vi "dynamic_roi_setting.vi"(8 "right_line_center":i32, 9 "left_line_center":i32, 10 "mid_far Descriptor":T2={"Global Rectangle"=[475, 215, 533, 216], "Contours"=[{"ID"=enum."External", "Type"=2, "Coordinates"=[530, 210, 580, 210]}]} {"Contours"."Type" items=["No Selection", "Point", "Line", "Rectangle", "Oval", "Polygon", "Freehand Region", "Annulus", "Unused2", "Unused3", "Broken Line", "Freehand Line", "Rotated Rectangle"]}, 11 "mid_near Descriptor":T2={"Global Rectangle"=[475, 216, 344, 218], "Contours"=[{"ID"=enum."External", "Type"=2, "Coordinates"=[200, 210, 250, 210]}]} {"Contours"."Type" items=["No Selection", "Point", "Line", "Rectangle", "Oval", "Polygon", "Freehand Region", "Annulus", "Unused2", "Unused3", "Broken Line", "Freehand Line", "Rotated Rectangle"]}) -> (2 "far_roi":T1, 3 "near_roi":T1)   [LabVIEW 2024]
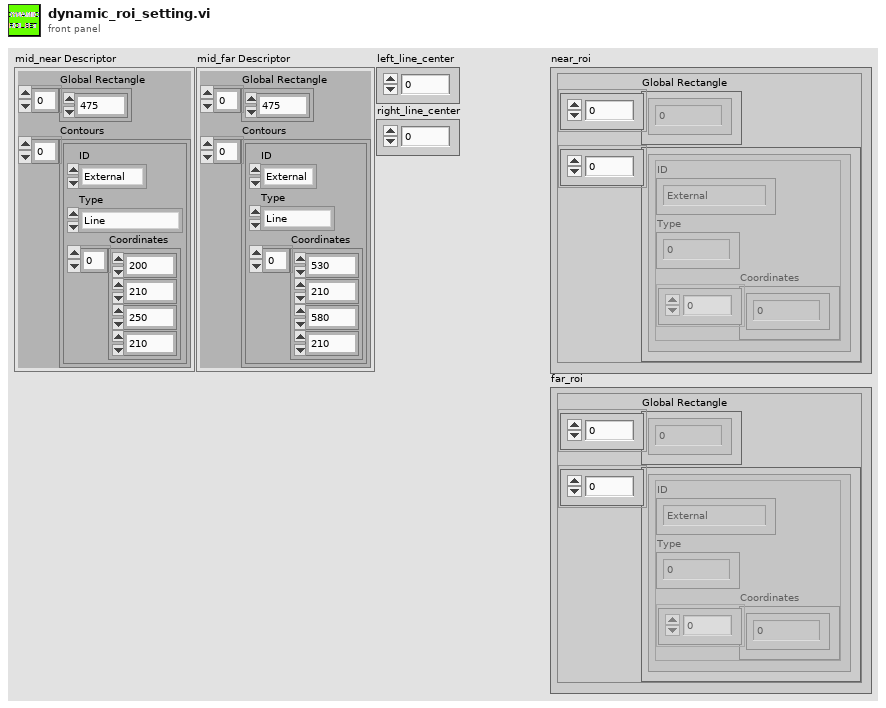
[diagram p1: front panel]
types:
  T1 = cluster{"Global Rectangle":i32[], "배열":cluster{"ID":enum32{"External", "Internal"}, "Type":u32, "Coordinates":i32[]}[]}
  T2 = cluster{"Global Rectangle":i32[], "Contours":cluster{"ID":enum32{"External", "Internal"}, "Type":u32, "Coordinates":i32[]}[]}
  T3 = cluster{"ID":enum32{"External", "Internal"}, "Type":u32, "Coordinates":i32[]}[]
  T4 = cluster{"ID":enum32{"External", "Internal"}, "Type":u32, "Coordinates":i32[]}
  T5 = cluster{"Global Rectangle":i32[], cluster{"ID":enum32{"External", "Internal"}, "Type":u32, "Coordinates":i32[]}[]}
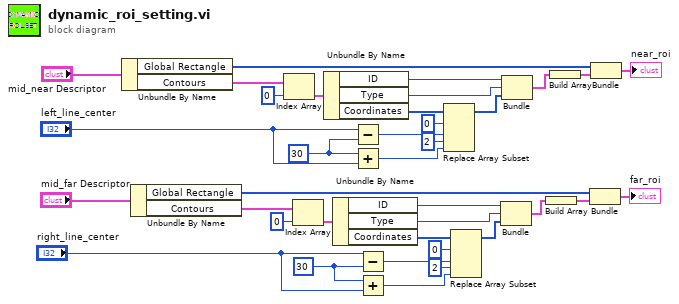
[diagram p0: block diagram]
diagram:
  w5 = 30
  w8 = 30
  n1 = Unbundle By Name("mid_near Descriptor") -> ("Global Rectangle"=w29:i32[], "Contours"=w36:T3)
  n2 = Unbundle By Name("mid_far Descriptor") -> ("Global Rectangle"=w18:i32[], "Contours"=w12:T3)
  n3 = Index Array(array=w36, index=0 ("인덱스")) -> (element=w34:T4)
  n4 = Index Array(array=w12, index=0 ("인덱스")) -> (element=w13:T4)
  n5 = Unbundle By Name(w34) -> ("ID"=w28:enum32{"External", "Internal"}, "Type"=w27:u32, "Coordinates"=w30:i32[])
  n6 = Unbundle By Name(w13) -> ("ID"=w19:enum32{"External", "Internal"}, "Type"=w20:u32, "Coordinates"=w17:i32[])
  n7 = Subtract(x="left_line_center", y=w8) -> (x-y=w7:i32)
  n8 = Add(x=w8, y="left_line_center") -> (x+y=w6:i32)
  n9 = Subtract(x="right_line_center", y=w5) -> (x-y=w4:i32)
  n10 = Add(x=w5, y="right_line_center") -> (x+y=w3:i32)
  n11 = Replace Array Subset(array=w30, new element #1=w7, index #1=0 ("인덱스"), new element #2=w6, index #2=2 ("인덱스")) -> (w26:i32[])
  n12 = Replace Array Subset(array=w17, new element #1=w4, index #1=0 ("인덱스"), new element #2=w3, index #2=2 ("인덱스")) -> (w21:i32[])
  n13 = Bundle("ID"=w19, "Type"=w20, "Coordinates"=w21) -> (w23:T4)  [unwired: 1 in]
  n14 = Bundle("ID"=w28, "Type"=w27, "Coordinates"=w26) -> (w24:T4)  [unwired: 1 in]
  n15 = Build Array(w23) -> (w22:T3)
  n16 = Build Array(w24) -> (w25:T3)
  n17 = Bundle("Global Rectangle"=w18, w22) -> (→"far_roi":T5)  [unwired: 1 in]
  n18 = Bundle("Global Rectangle"=w29, w25) -> (→"near_roi":T5)  [unwired: 1 in]
